vi "Write Barcode.vi"(8 "error in (no error)":errorcluster, 9 "data":variant, 10 "String":string, 11 "URL":string) -> (0 "error out":errorcluster, 1 "code":string, 2 "Log":string, 3 "ok?":bool)   [LabVIEW 2012]
uses:
  write_String.vi
  write_Num.vi
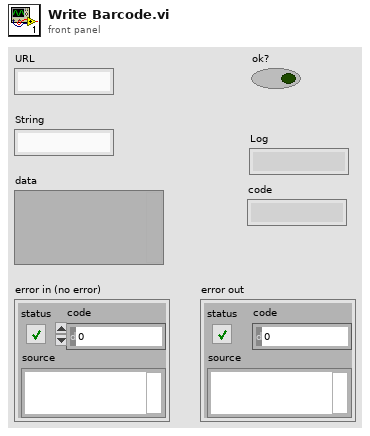
[diagram p1: front panel]
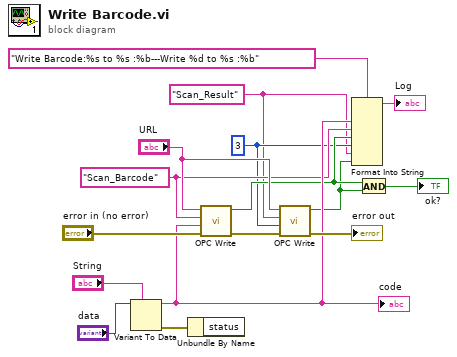
[diagram p0: block diagram]
diagram:
  w4 = 3 ("Value")
  w3 = "Scan_Result" ("Address")
  w6 = "Scan_Barcode" ("Address")
  n1 = Variant To Data(type="String", Variant="data") -> (data=w7:string, error out=w12:errorcluster)  [unwired: 1 in]
  "code" <- w7
  n2 = Unbundle By Name(w12) -> ()  [unwired: 1 out]
  n3 = call-poly "OPC Write.vi"("错误输入（无错误）"="error in (no error)", "Value"=w7, "Address"=w6, "URL"="URL") -> ("error out"=w15:errorcluster, "ok?"=w5:bool)  [unwired: 6 in]
  n4 = call-poly "OPC Write.vi"("错误输入（无错误）"=w15, "Value"=w4, "Address"=w3, "URL"="URL") -> ("error out"=→"error out":errorcluster, "ok?"=w2:bool)  [unwired: 6 in]
  n5 = Format Into String(format string="Write Barcode:%s to %s :%b---Write %d to %s :%b", w7, w6, w5, w4, w3, w2) -> (resulting string=→"Log":string)  [unwired: 2 in, 1 out]
  n6 = And(x=w5, y=w2) -> (x .and. y?=→"ok?":bool)
